vi "clone.vi"(0 "reference":refnum<class "NoteNode.lvclass">, 5 "error in (no error)":errorcluster) -> (14 "reference out":refnum<class "NoteNode.lvclass">, 15 "clonedNote":refnum<class "AbstractNode.lvclass">, 19 "error out":errorcluster)   [LabVIEW 2020, in "NoteNode.lvclass"]
doc: "public Object clone()"
uses:
  <resource>/Framework/Providers/Open_GDS/UML/NoteNode_class/NoteNode.lvclass
  C:/Program Files (x86)/National Instruments/LabVIEW 2020/resource/Framework/Providers/Open_GDS/UML/RectangularNode_class/RectangularNode.lvclass
  C:/Program Files (x86)/National Instruments/LabVIEW 2020/resource/Framework/Providers/Open_GDS/UML/AbstractNode_class/AbstractNode.lvclass
  <resource>/Framework/Providers/Open_GDS/UML/AbstractNode_class/AbstractNode.lvclass
  <resource>/Framework/Providers/Open_GDS/UML/MultiLineString_class/MultiLineString.lvclass
  <resource>/Framework/Providers/Open_GDS/UML/RectangularNode_class/RectangularNode.lvclass
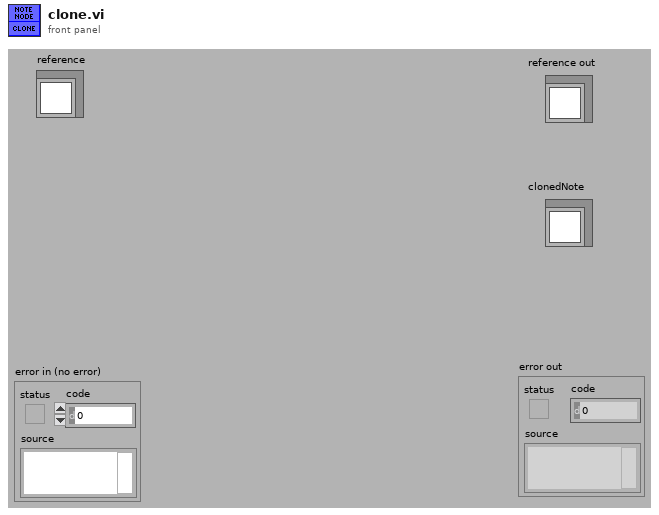
[diagram p1: front panel]
types:
  T1 = typedef "RectangularNode.lvclass/ObjectAttributes.ctl" = cluster{"bounds":T2}
  T2 = typedef "Rectangle Rectangle2D.ctl" = cluster{"x":dbl, "y":dbl, "width":dbl, "height":dbl}
  T3 = typedef "NoteNode.lvclass/ObjectAttributes.ctl" = cluster{"DEFAULT_WIDTH":i32, "DEFAULT_HEIGHT":i32, "DEFAULT_COLOR":u32, "FOLD_X":i32, "FOLD_Y":i32, "color":u32, "text":refnum<class "MultiLineString.lvclass">, "pointNodes":refnum<class "AbstractNode.lvclass">[]}
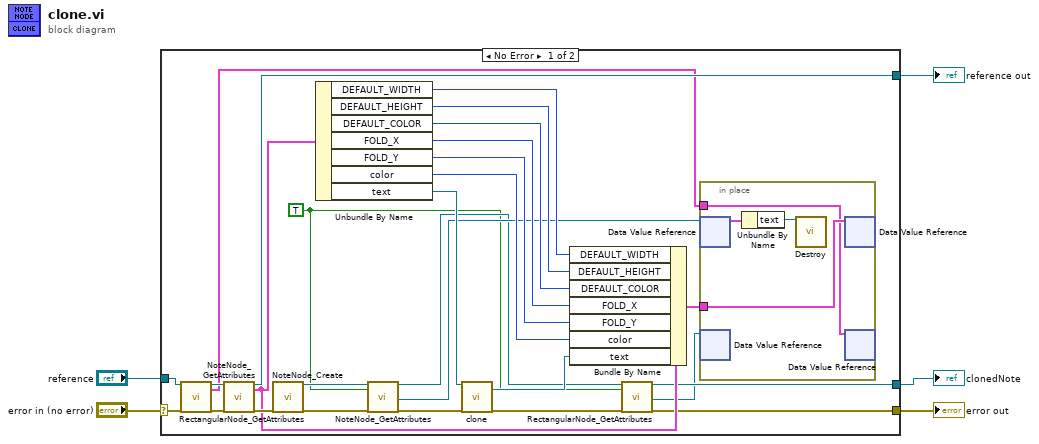
[diagram p0: block diagram]
diagram:
  n1 = case shown="No Error" "error in (no error)" {
    selector: "error in (no error)" -> [w31 w37]
    tunnel: "reference" -> [w13 w38]
    tunnel: [w11 w37] -> w4
    tunnel: [w32 w38] -> w3
    tunnel: [w9 _] -> w1
    frame No Error {
      w7 = TRUE ("OnlyGetDvrReference(False)")
      n2 = call <resource>:"RectangularNode_GetAttributes.vi"("reference in"=w13, "error in (no error)"=w31) -> ("reference out"=w12:refnum<class "NoteNode.lvclass">, "Data"=w6:T1, "error out"=w14:errorcluster)  [unwired: 14 in, 1 out]
      n3 = call <resource>:"NoteNode_GetAttributes.vi"("reference in"=w12, "error in (no error)"=w14) -> ("reference out"=w32:refnum<class "NoteNode.lvclass">, "Data"=w18:T3, "error out"=w19:errorcluster)  [unwired: 1 in, 14 out]
      n4 = call <resource>:"NoteNode_Create.vi"("error in (no error)"=w19) -> ("reference out"=w20:refnum<class "NoteNode.lvclass">, "error out"=w30:errorcluster)  [unwired: 17 in]
      n5 = Unbundle By Name(w18) -> ("DEFAULT_WIDTH"=w29:i32, "DEFAULT_HEIGHT"=w28:i32, "DEFAULT_COLOR"=w27:u32, "FOLD_X"=w26:i32, "FOLD_Y"=w25:i32, "color"=w21:u32, "text"=w24:refnum<class "MultiLineString.lvclass">)
      n6 = call <resource>:"NoteNode_GetAttributes.vi"("reference in"=w20, "OnlyGetDvrReference(False)"=w7, "error in (no error)"=w30) -> ("reference out"=w10:refnum<class "NoteNode.lvclass">, "DataRef"=w16:refnum<data-value>, "error out"=w23:errorcluster)  [unwired: 13 in, 1 out]
      n7 = call-dynamic "clone.vi"("reference"=w24, "error in (no error)"=w23) -> ("clonedMultiLineString"=w22:refnum<class "MultiLineString.lvclass">, "error out"=w17:errorcluster)  [unwired: 15 in, 1 out]
      n8 = Bundle By Name(cluster=w18, "DEFAULT_WIDTH"=w29, "DEFAULT_HEIGHT"=w28, "DEFAULT_COLOR"=w27, "FOLD_X"=w26, "FOLD_Y"=w25, "color"=w21, "text"=w22) -> (w15:T3)
      n9 = call <resource>:"RectangularNode_GetAttributes.vi"("reference in"=w10, "OnlyGetDvrReference(False)"=w7, "error in (no error)"=w17) -> ("reference out"=w9:refnum<class "NoteNode.lvclass">, "DataRef"=w8:refnum<data-value>, "error out"=w11:errorcluster)  [unwired: 13 in, 1 out]
      n10 = in-place {
        in-place-border: w15 -> [w36]
        in-place-border: w6 -> [w33]
        n11 = in-place-dvr #1(w16) -> (w34:T3)  [unwired: 1 out]
        n12 = in-place-dvr #2(w8) -> ()  [unwired: 2 out]
        n13 = Unbundle By Name(w34) -> ("text"=w35:refnum<class "MultiLineString.lvclass">)
        n14 = call-dynamic "Destroy.vi"("reference"=w35) -> ()  [unwired: 17 in, 2 out]
        n15 = in-place-dvr #1(w36) -> ()  [unwired: 2 out]
        n16 = in-place-dvr #2(w33) -> ()  [unwired: 2 out]
      }
    }
    frame Error {
    }
  }
  "reference out" <- w3
  "error out" <- w4
  "clonedNote" <- w1
